vi "Settings Dialog.vi"(7 "Host":T1={"NI Software"=[{"ID"="ni-datasocket", "Version"="21.0.0.49352-0+f200"}, {"ID"="ni-vipm", "Version"="21.1.0.49472-0+f320"}, {"ID"="ni-labview-2021-core-x86-en", "Version"="21.1.2.49154-0+f2"}, {"ID"="ni-labview-2021-community-x86", "Version"="21.1.0.49478-0+f326"}, {"ID"="ni-labview-2021-database-toolkit-x86", "Version"="21.0.0.49154-0+f2"}, {"ID"="ni-labview-2021-datafinder-runtime-x86", "Version"="21.0.0.49153-0+f1"}, {"ID"="ni-labview-2021-datafinder-connectivity-x86", "Version"="21.0.0.49152-0+f0"}, {"ID"="ni-labview-2021-linx-toolkit-x86", "Version"="21.1.0.49152-0+f0"}, {"ID"="ni-labview-2021-report-generation-toolkit-x86", "Version"="21.0.0.49154-0+f2"}, {"ID"="ni-labview-2019-runtime-engine-x86", "Version"="19.1.5.49152-0+f0"}, {"ID"="ni-labview-2020-runtime-engine-x86", "Version"="20.1.1.49157-0+f5"}, {"ID"="ni-labview-2021-runtime-engine-x86", "Version"="21.1.2.49154-0+f2"}, {"ID"="ni-cvi-dotnet", "Version"="20.0.0.49152-0+f0"}, {"ID"="ni-cvi-analysis", "Version"="20.0.0.49152-0+f0"}, {"ID"="ni-cvi-networkstreams", "Version"="20.0.0.49152-0+f0"}, {"ID"="ni-cvi-network-variable", "Version"="20.0.0.49152-0+f0"}, {"ID"="ni-cvi-runtime-engine", "Version"="20.0.2.49152-0+f0"}, {"ID"="ni-cvi-rte", "Version"="20.0.2.49152-0+f0"}, {"ID"="ni-cvi-tdms", "Version"="20.0.1.49152-0+f0"}, {"ID"="mgi-solution-explorer", "Version"="2.5.0-53"}, {"ID"="ni-certificates", "Version"="21.5.0.49170-0+f18"}, {"ID"="ni-dataplugins-aop5", "Version"="19.5.0.7555-0+f2"}, {"ID"="ni-distributed-system-manager-2021", "Version"="21.0.0.49488-0+f336"}, {"ID"="ni-hardware-configuration-importer", "Version"="8.4.0.49152-0+f0"}, {"ID"="ni-labview-command-line-interface-x86", "Version"="4.0.0.49152-0+f0"}, {"ID"="ni-license-manager", "Version"="21.3.1.49163-0+f11"}, {"ID"="ni-max", "Version"="21.5.0.49391-0+f239"}, {"ID"="ni-package-manager", "Version"="23.0.0.49276-0+f124"}, {"ID"="ni-syscfg-dotnet-runtime", "Version"="21.5.0.49392-0+f240"}, {"ID"="ni-syscfg-runtime", "Version"="21.5.0.49392-0+f240"}, {"ID"="ni-syscfg-labview-2021-support-x86", "Version"="21.5.0.49392-0+f240"}, {"ID"="ni-system-webserver", "Version"="21.5.0.49152-0+f0"}, {"ID"="ni-update-service", "Version"="21.0.0.49243-0+f91"}, {"ID"="ni-usi-core", "Version"="21.5.0.49152-0+f0"}, {"ID"="ni-webserver", "Version"="21.3.0.49152-0+f0"}, {"ID"="ni-webservices-amqp-deployment-support-x86", "Version"="21.5.0.49152-0+f0"}, {"ID"="ni-webservices-amqp-labview-2021-support-x86", "Version"="21.5.0.49152-0+f0"}, {"ID"="ni-web-based-configuration", "Version"="21.5.0.49392-0+f240"}, {"ID"="ni-visa-runtime", "Version"="21.5.0.49252-0+f100"}, {"ID"="ni-variable-engine", "Version"="21.0.0.49350-0+f198"}], "IO Devices"=[]}, 8 "error in (no error)":errorcluster, 11 "Settings in":T13={"IO"={"Channel Settings"=[{"Name"="sim1", "Terminal Information"={"IO Device"=enum."none", "Channel"=0, "Sensor Type"=enum."Voltage"}, "Calibration Information"={"Excitation Voltage"=1.0, "Calibration Factor"=1.0, "Zero Value"=0.0, "Calibration Formula"="y = (x-x0) / (Ve * CF)", "Units"=""}}, {"Name"="sim2", "Terminal Information"={"IO Device"=enum."none", "Channel"=1, "Sensor Type"=enum."Voltage"}, "Calibration Information"={"Excitation Voltage"=1.0, "Calibration Factor"=1.0, "Zero Value"=0.0, "Calibration Formula"="(x-x0) / (Ve * CF)", "Units"=""}}, {"Name"="sim3", "Terminal Information"={"IO Device"=enum."none", "Channel"=2, "Sensor Type"=enum."Voltage"}, "Calibration Information"={"Excitation Voltage"=1.0, "Calibration Factor"=1.0, "Zero Value"=0.0, "Calibration Formula"="y = (x-x0) / (Ve * CF)", "Units"=""}}, {"Name"="sim4", "Terminal Information"={"IO Device"=enum."none", "Channel"=3, "Sensor Type"=enum."Voltage"}, "Calibration Information"={"Excitation Voltage"=1.0, "Calibration Factor"=1.0, "Zero Value"=0.0, "Calibration Formula"="(x-x0) / (Ve * CF)", "Units"=""}}], "Sensor Intervals"=[{"Interval"=enum."1 second", "Count"=1}], "Sensor Token"={"Next reading in ms"=0, "Interval Index"=0, "Interval Occurrence"=0}, "IO Context"={"Active Plugin"="", "API"=enum."Simulated", "API Wire"=variant}}, "Log"={"Path"=path "C:/dev/mux/git/github/lv-daq-app-template/data_log.csv", "Spreadsheet"=refnum, "Mode"=enum."Append"}, "Debug"={"Messages"=refnum}, "Graph Settings"={"Small Scale Max"=0.0, "Large Scale Max"=0.0, "Large Scale Threshold"=0.0}}) -> (0 "error out":errorcluster, 1 "Cancelled?":bool=TRUE, 3 "Settings out":T13={"IO"={"Channel Settings"=[{"Name"="sim1", "Terminal Information"={"IO Device"=enum."none", "Channel"=0, "Sensor Type"=enum."Voltage"}, "Calibration Information"={"Excitation Voltage"=1.0, "Calibration Factor"=1.0, "Zero Value"=0.0, "Calibration Formula"="y = (x-x0) / (Ve * CF)", "Units"=""}}, {"Name"="sim2", "Terminal Information"={"IO Device"=enum."none", "Channel"=1, "Sensor Type"=enum."Voltage"}, "Calibration Information"={"Excitation Voltage"=1.0, "Calibration Factor"=1.0, "Zero Value"=0.0, "Calibration Formula"="(x-x0) / (Ve * CF)", "Units"=""}}, {"Name"="sim3", "Terminal Information"={"IO Device"=enum."none", "Channel"=2, "Sensor Type"=enum."Voltage"}, "Calibration Information"={"Excitation Voltage"=1.0, "Calibration Factor"=1.0, "Zero Value"=0.0, "Calibration Formula"="y = (x-x0) / (Ve * CF)", "Units"=""}}, {"Name"="sim4", "Terminal Information"={"IO Device"=enum."none", "Channel"=3, "Sensor Type"=enum."Voltage"}, "Calibration Information"={"Excitation Voltage"=1.0, "Calibration Factor"=1.0, "Zero Value"=0.0, "Calibration Formula"="(x-x0) / (Ve * CF)", "Units"=""}}], "Sensor Intervals"=[{"Interval"=enum."1 second", "Count"=1}], "Sensor Token"={"Next reading in ms"=0, "Interval Index"=0, "Interval Occurrence"=0}, "IO Context"={"Active Plugin"="", "API"=enum."Simulated", "API Wire"=variant}}, "Log"={"Path"=path "C:/dev/mux/git/github/lv-daq-app-template/data_log.csv", "Spreadsheet"=refnum, "Mode"=enum."Append"}, "Debug"={"Messages"=refnum}, "Graph Settings"={"Small Scale Max"=0.0, "Large Scale Max"=0.0, "Large Scale Threshold"=0.0}})   [LabVIEW 2021, in "Settings.lvlib"]
doc: "Dialog for selecting user specified settings."
uses:
  Settings.lvlib
  Settings.ctl
  Acquisition/Hardware Configuration.ctl
  Acquisition/Channel Settings.ctl
  Acquisition/IO Device.ctl
  Acquisition/Sensor Type.ctl
  Interval Timer/Repeat Interval.ctl
  Interval Timer/Interval Length.ctl
  Interval Timer/Interval Token.ctl
  Acquisition/IO Context.ctl
  Acquisition/IO API.ctl
  Logging/Logging Configuration.ctl
  Logging/Logging Mode.ctl
  Diagnostics/Diagnostics Configuration.ctl
  controls/Graph Settings.ctl
  Acquisition/Host Resources.ctl
  Acquisition/Host Software Package.ctl
  Acquisition/Host IO Resource.ctl
  Logging/Logging.lvlib
  Acquisition/Acquisition.lvlib
  Diagnostics/Diagnostics.lvlib
  Interval Timer/Interval Timer.lvlib
panel:
  in  "IO tab control":T4(tab)
  in  "Channel Settings":T7(array[cluster])
  in  "Calibration Settings":T8(array[cluster])
  in  "New x0 Button":bool
  out "x0":dbl=nan
  out "CF":dbl=nan
  out "Vex":dbl=nan
  out "Preview Chart":waveform(dbl)(graph)={"t0"=timestamp(3763062488.961019 s since 1904-01-01), "dt"=1.0, "Y"=[3.134800048306457], "attributes"=variant("NI_ChannelName"=variant(string "sim1"))}
  in  "Channel to Preview":string(combo)
  in  "Stop Preview Button":bool
  in  "Start Preview Button":bool
  in  "Active Plugin":string(combo)
  in  "Graph settings":T9
  in  "Sensor Intervals":T10[](array[typedef])=[{"Interval"=enum."1 second", "Count"=1}]
  out "Host out":T1
  in  "Log File tab control":T12(tab)=enum."Append to existing log"
  in  "Refresh Button":bool
  in  "New log file path":path=path "C:/dev/mux/git/github/lv-daq-app-template/data_log.csv"
  in  "Existing log file path":string="C:\\dev\\mux\\git\\github\\lv-daq-app-template\\data_log.csv"
  in  "Autoname new log path":string="C:\\dev\\mux\\git\\github\\lv-daq-app-template\\data_log.csv"
  in  "Cancel Button":bool
  in  "OK Button":bool
  # "Non visible portion of dialog (needed for connector pane)."
  # "Method: (x-x0) / (Ve * CF)"
  # "Method: (x-x0) / (Ve * CF)"
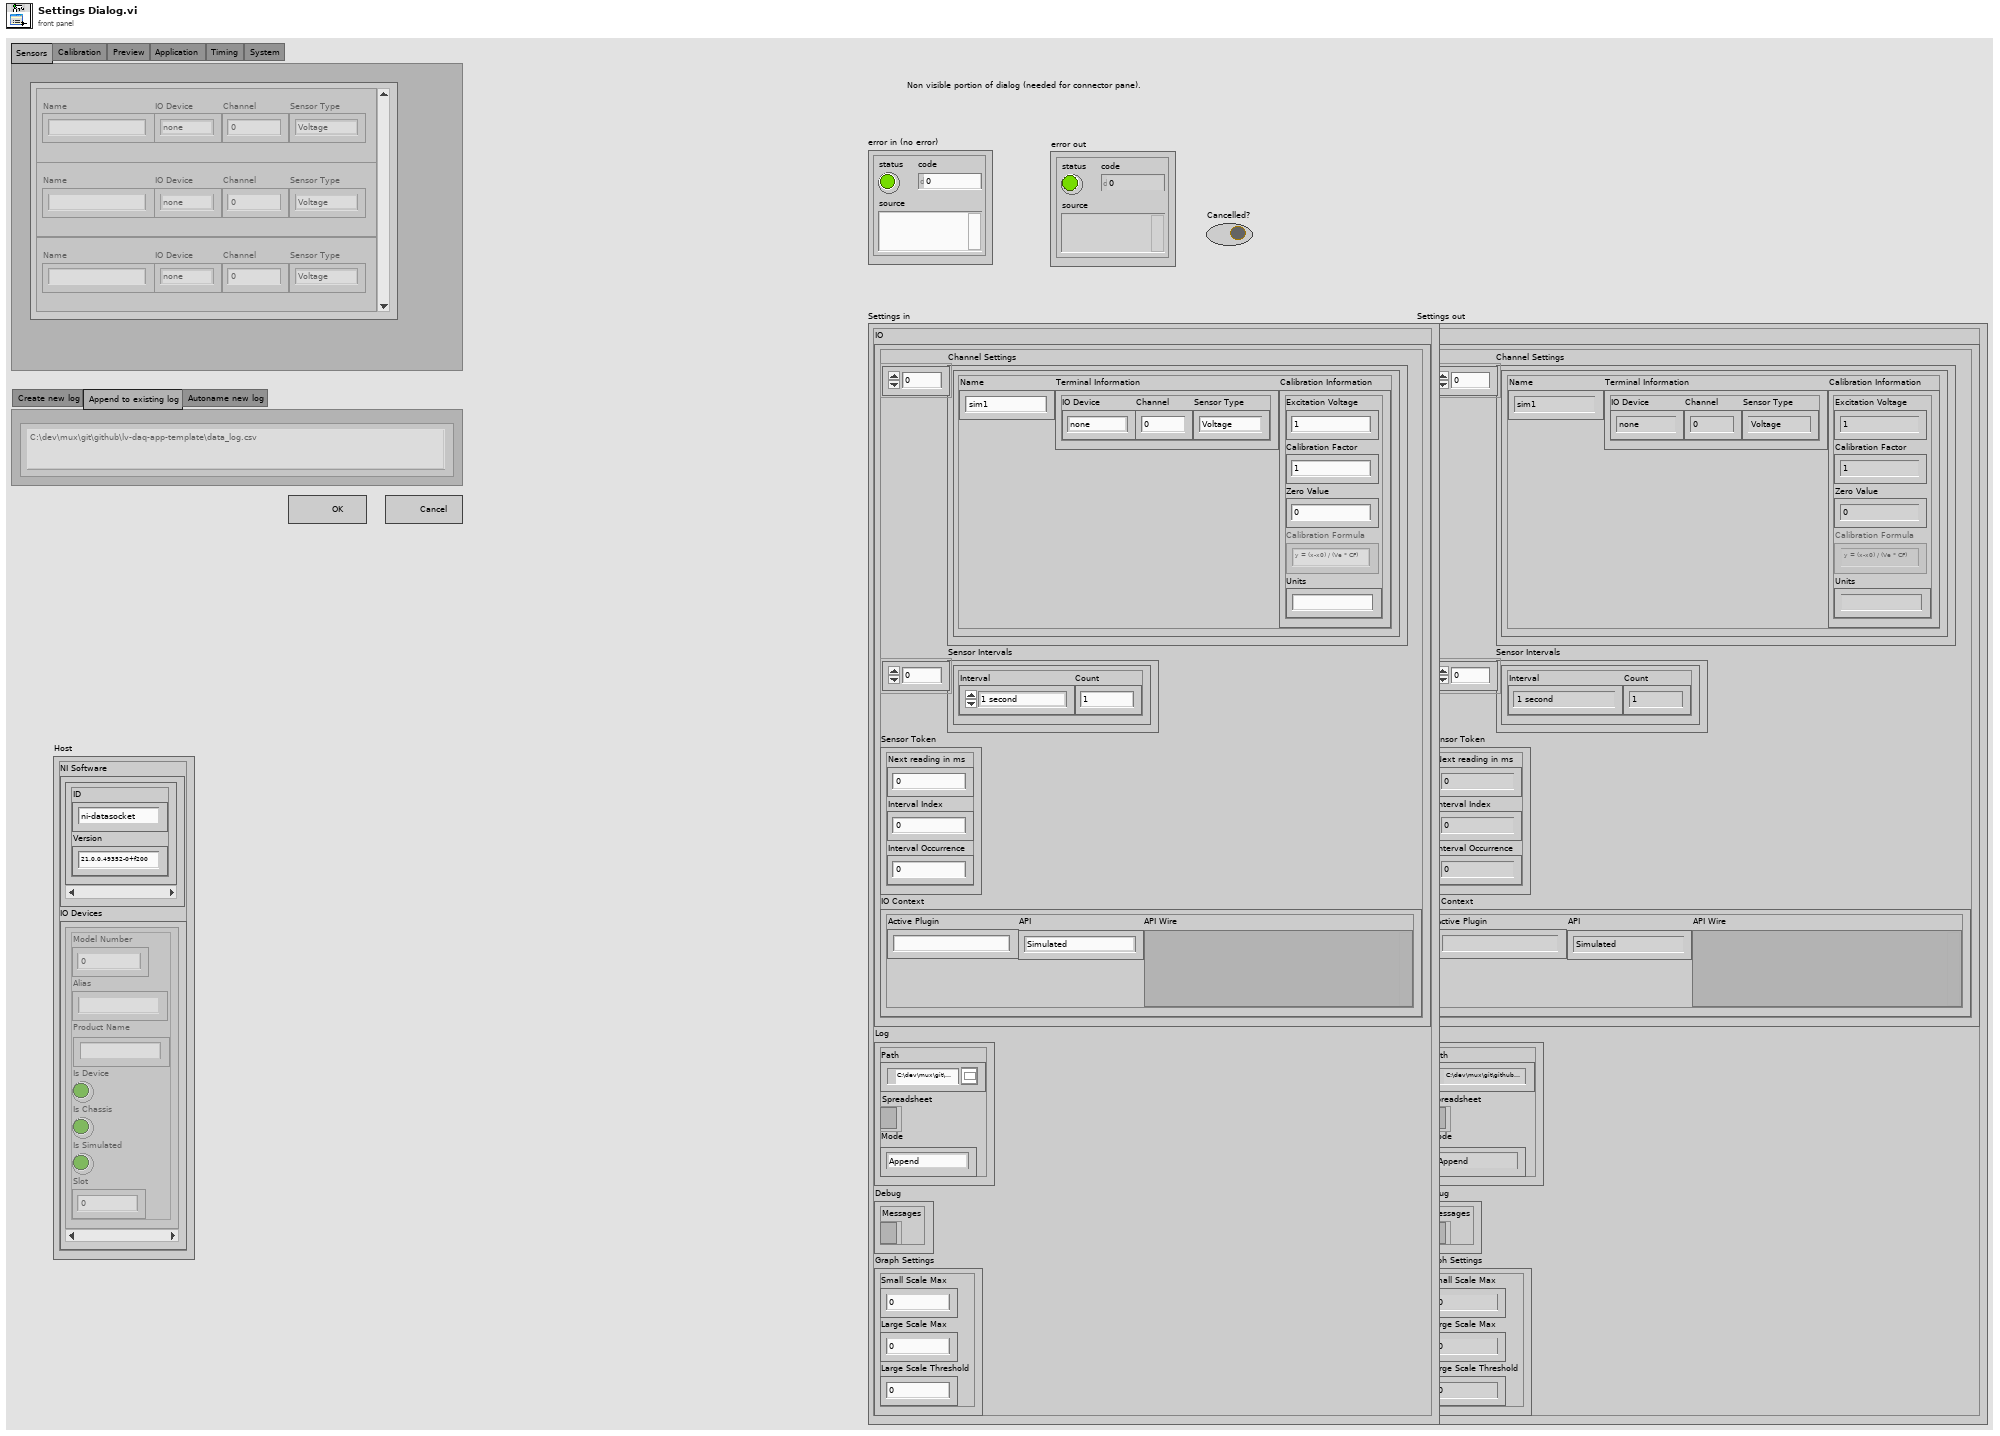
[diagram p1: front panel]
types:
  T1 = typedef "Acquisition.lvlib/Host Resources.ctl" = cluster{"NI Software":T2[], "IO Devices":T3[]}
  T2 = typedef "Acquisition.lvlib/Host Software Package.ctl" = cluster{"ID":string, "Version":string}
  T3 = typedef "Acquisition.lvlib/Host IO Resource.ctl" = cluster{"Model Number":u32, "Alias":string, "Product Name":string, "Is Device":bool, "Is Chassis":bool, "Is Simulated":bool, "Slot":i32}
  T4 = enum32{"Sensors", "Calibration", "Preview", "Application", "Timing", "System"}
  T5 = typedef "Acquisition.lvlib/IO Device.ctl" = enum16{"none", "9219", "9401"}
  T6 = typedef "Acquisition.lvlib/Sensor Type.ctl" = enum16{"Voltage", "Load", "Pressure", "Encoder"}
  T7 = cluster{"Name":string, "Terminal Information":cluster{"IO Device":T5, "Channel":i32, "Sensor Type":T6}}[]
  T8 = cluster{"Name":string, "Calibration Information":cluster{"Excitation":dbl, "Cal. Factor":dbl, "Zero Value":dbl, "Units":string}}[]
  T9 = cluster{"Small Scale Maximum":dbl, "Large Scale Threshold":dbl, "Large Scale Maximum":dbl}
  T10 = typedef "Interval Timer.lvlib/Repeat Interval.ctl" = cluster{"Interval":T11, "Count":i32}
  T11 = typedef "Interval Timer.lvlib/Interval Length.ctl" = enum16{"Manual control", "1 second", "10 seconds", "30 seconds", "60 seconds", "600 seconds", "1200 seconds", "3600 seconds"}
  T12 = enum32{"Create new log", "Append to existing log", "Autoname new log"}
  T13 = typedef "Settings.lvlib/Settings.ctl" = cluster{"IO":T14, "Log":T19, "Debug":T21, "Graph Settings":T22}
  T14 = typedef "Acquisition.lvlib/Hardware Configuration.ctl" = cluster{"Channel Settings":T15[], "Sensor Intervals":T10[], "Sensor Token":T16, "IO Context":T17}
  T15 = typedef "Acquisition.lvlib/Channel Settings.ctl" = cluster{"Name":string, "Terminal Information":cluster{"IO Device":T5, "Channel":i32, "Sensor Type":T6}, "Calibration Information":cluster{"Excitation Voltage":dbl, "Calibration Factor":dbl, "Zero Value":dbl, "Calibration Formula":string, "Units":string}}
  T16 = typedef "Interval Timer.lvlib/Interval Token.ctl" = cluster{"Next reading in ms":u32, "Interval Index":i32, "Interval Occurrence":i32}
  T17 = typedef "Acquisition.lvlib/IO Context.ctl" = cluster{"Active Plugin":string, "API":T18, "API Wire":variant}
  T18 = typedef "Acquisition.lvlib/IO API.ctl" = enum16{"Simulated", "DAQmx"}
  T19 = typedef "Logging.lvlib/Logging Configuration.ctl" = cluster{"Path":path, "Spreadsheet":refnum<file>, "Mode":T20}
  T20 = typedef "Logging.lvlib/Logging Mode.ctl" = enum16{"Overwrite", "Append", "Create New"}
  T21 = typedef "Diagnostics.lvlib/Diagnostics Configuration.ctl" = cluster{"Messages":refnum<file>}
  T22 = typedef "Graph Settings.ctl" = cluster{"Small Scale Max":dbl, "Large Scale Max":dbl, "Large Scale Threshold":dbl}
  T23 = cluster{"Name":string, "Calibration Information":cluster{"Excitation Voltage":dbl, "Calibration Factor":dbl, "Zero Value":dbl, "Units":string}}[]
  T24 = typedef "Acquisition.lvlib/Acquired Data.ctl" = cluster{"Waveform Array":waveform(dbl)[]}
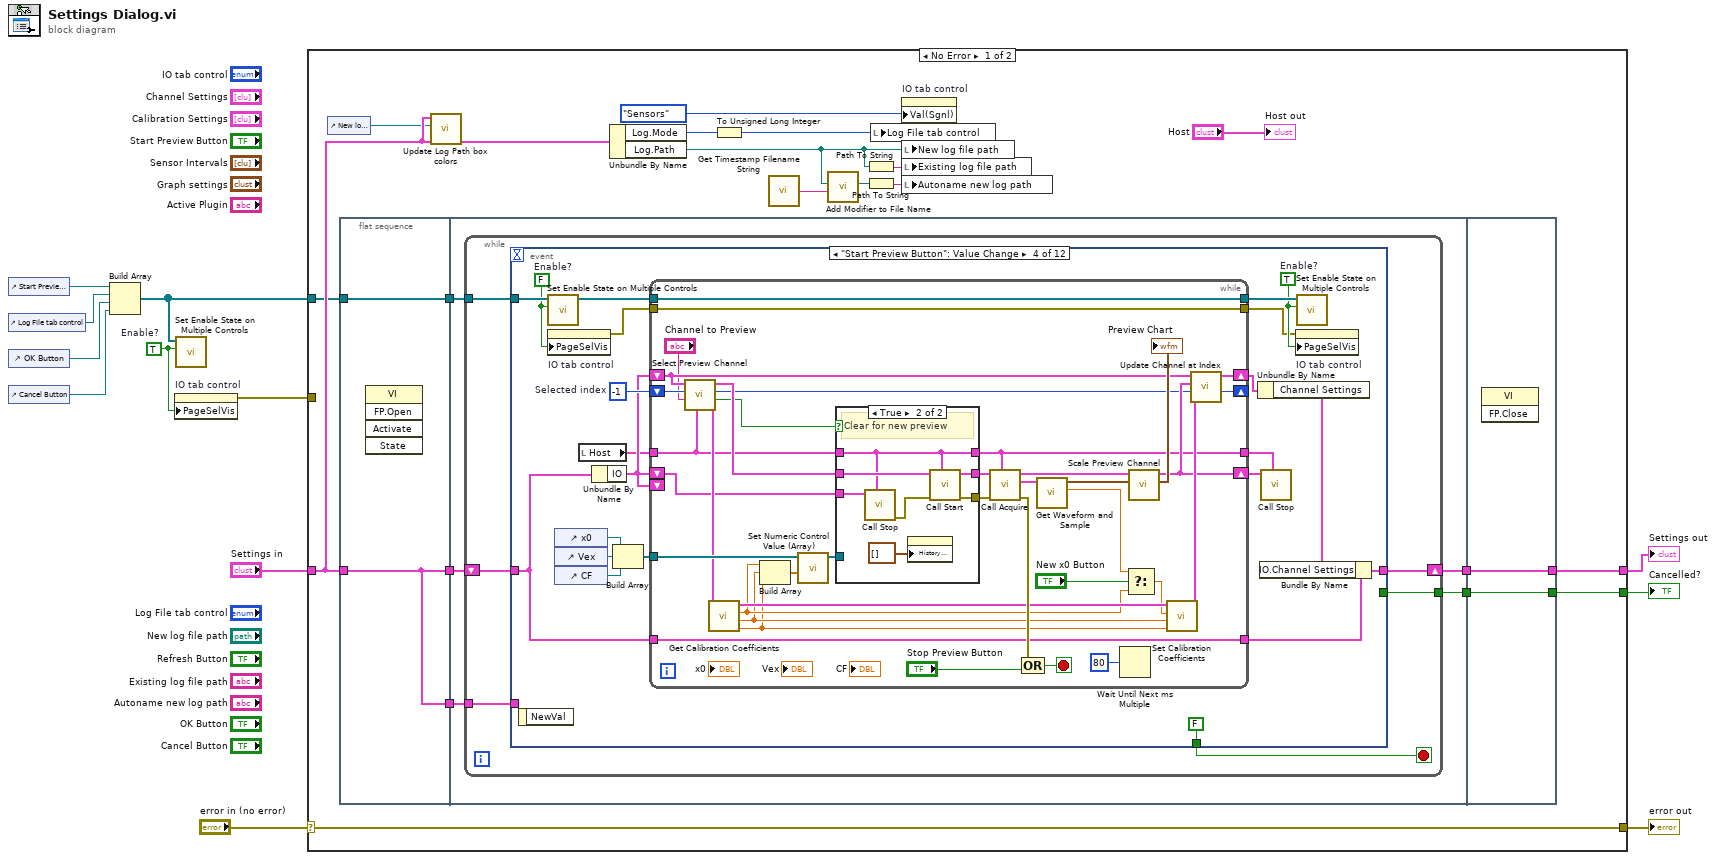
[diagram p0: block diagram]
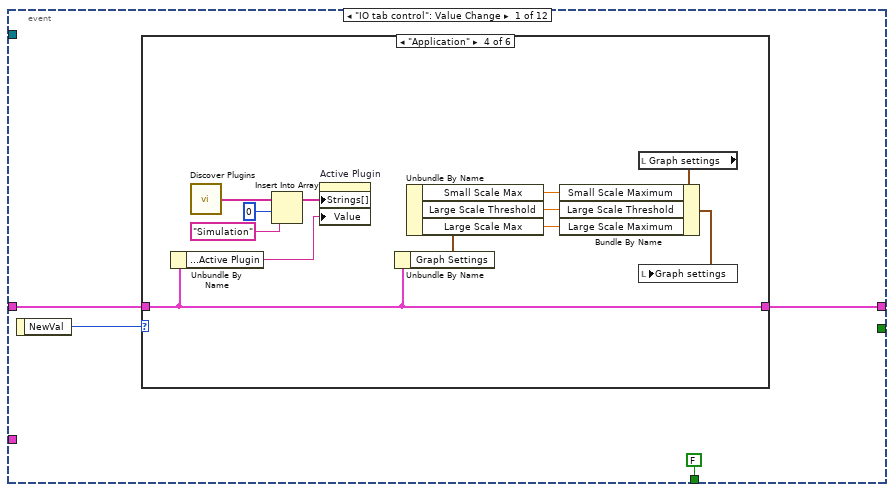
[diagram p2: hidden frame]
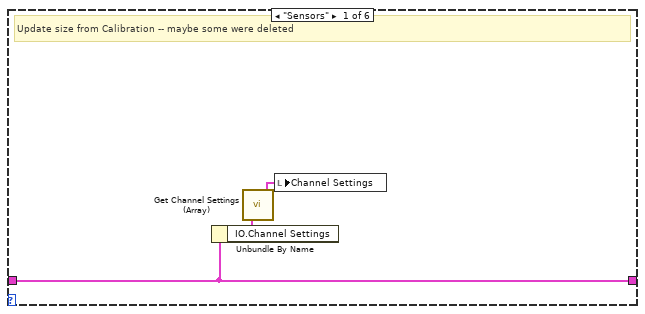
[diagram p3: hidden frame]
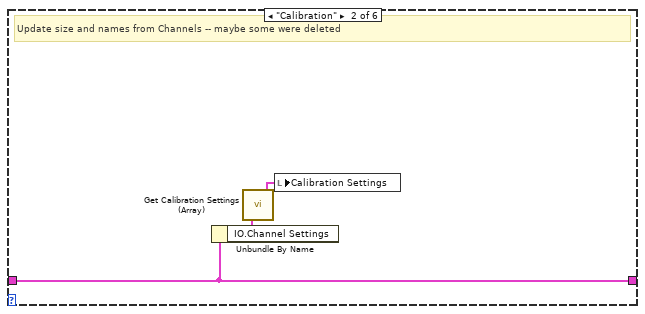
[diagram p4: hidden frame]
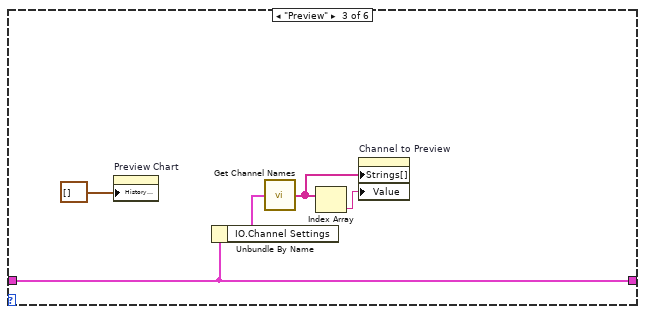
[diagram p5: hidden frame]
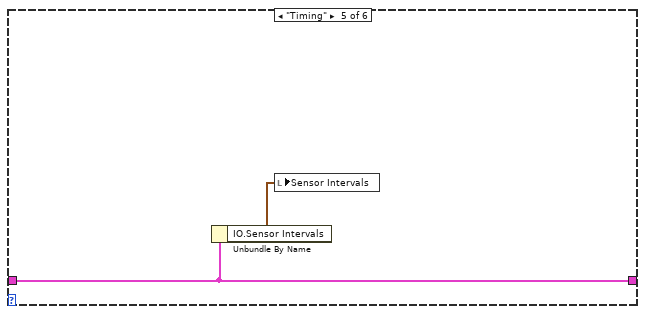
[diagram p6: hidden frame]
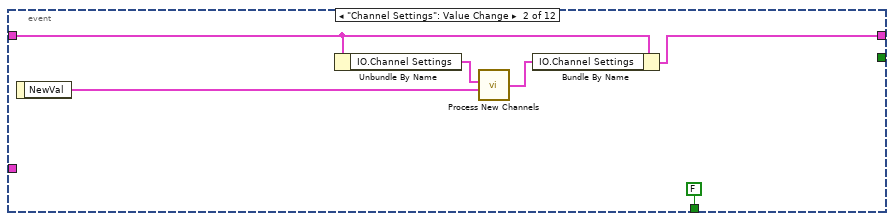
[diagram p8: hidden frame]
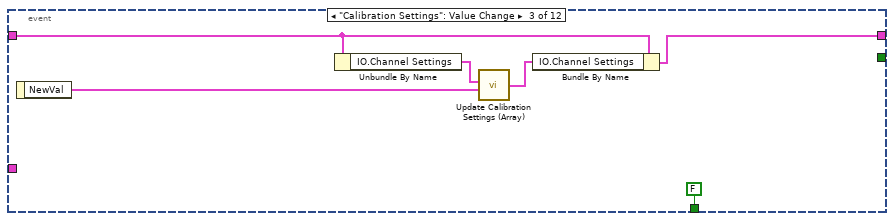
[diagram p9: hidden frame]
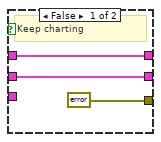
[diagram p10: hidden frame]
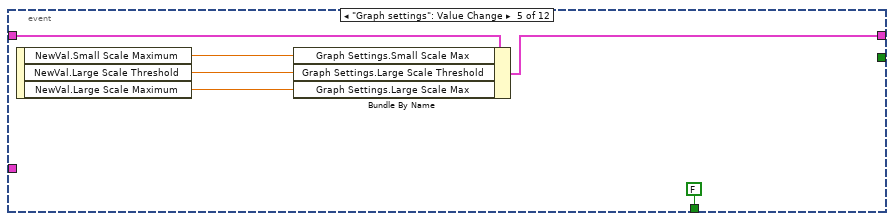
[diagram p11: hidden frame]
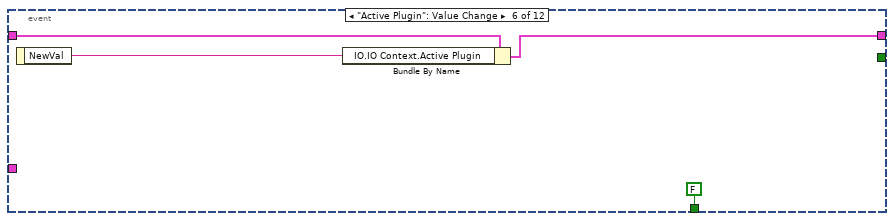
[diagram p12: hidden frame]
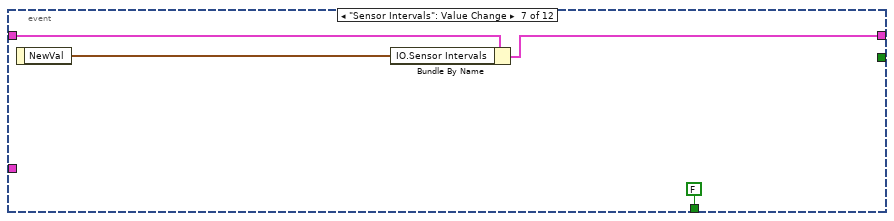
[diagram p13: hidden frame]
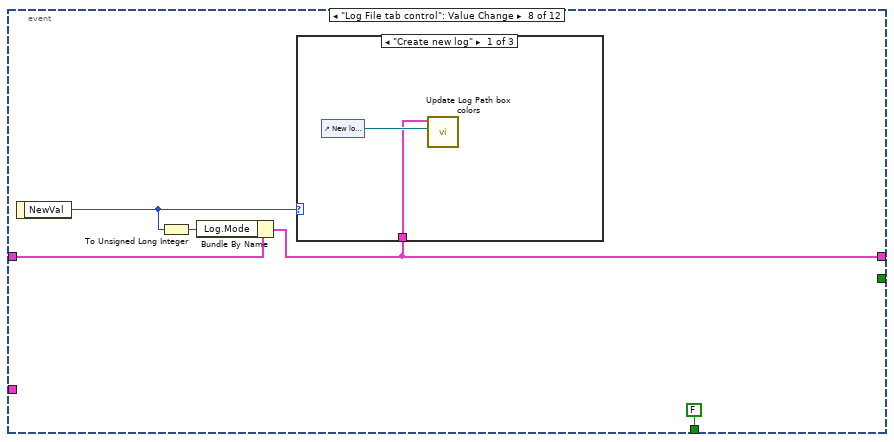
[diagram p14: hidden frame]
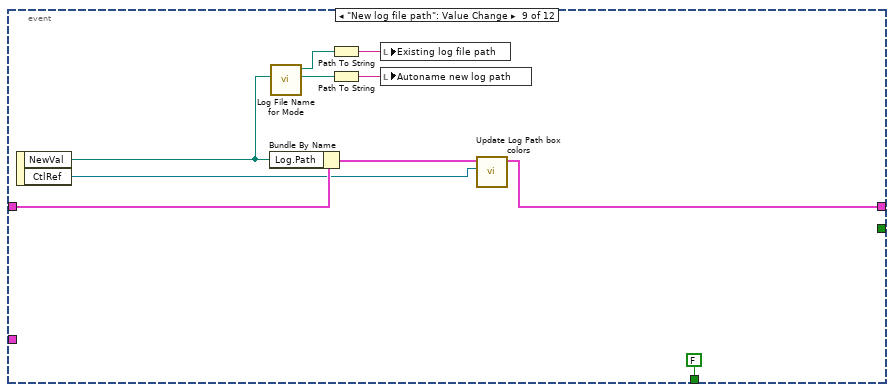
[diagram p17: hidden frame]
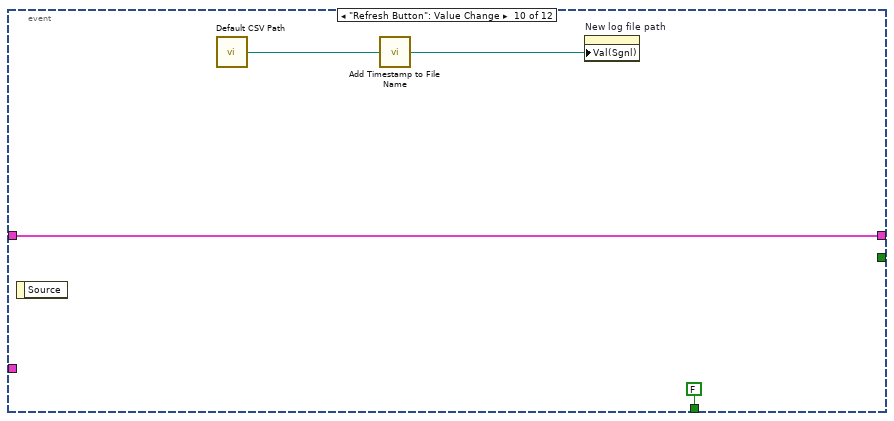
[diagram p18: hidden frame]
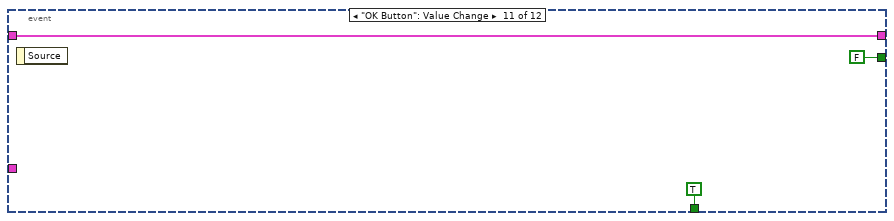
[diagram p19: hidden frame]
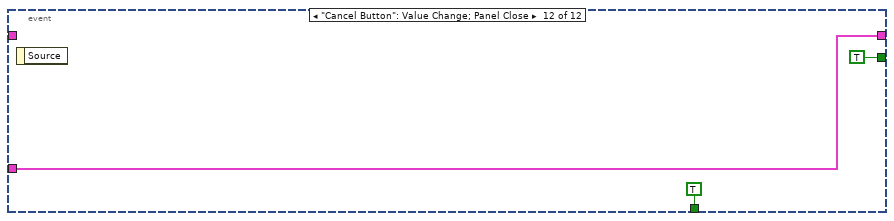
[diagram p20: hidden frame]
diagram:
  w2 = TRUE  # Enable?
  n1 = control-ref of="Start Preview Button"() -> (w7:refnum<vi>)
  n2 = control-ref of="Log File tab control"() -> (w6:refnum<vi>)
  n3 = control-ref of="OK Button"() -> (w5:refnum<vi>)
  n4 = control-ref of="Cancel Button"() -> (w4:refnum<vi>)
  n5 = Build Array(w7, w6, w5, w4) -> (w3:refnum<vi>[])
  n6 = property on="IO tab control" class="TabCtl (strict)"("PageSelVis"=w2) -> (error out=w1:errorcluster)  [unwired: 2 in, 1 out]
  n7 = call "Set Enable State on Multiple Controls.vi"("Enable?"=w2, "Controls"=w3) -> ()  [unwired: 9 in, 1 out]
  n8 = case shown="No Error" "error in (no error)" {
    selector: "error in (no error)" -> [w32 w202]
    tunnel: [w32 w202] -> w11
    tunnel: "Settings in" -> [w25 w201]
    tunnel: [w31 w201] -> w9
    tunnel: [w26 TRUE ("UI Refresh Needed?")] -> w8
    tunnel: w3 -> [w22 _]
    tunnel: w1 -> [_ _]
    frame No Error {
      n9 = control-ref of="New log file path"() -> (w24:refnum<vi>)
      n10 = flat-sequence {
        tunnel: w25 -> [w33]
        tunnel: [w33] -> w30
        tunnel: [w34] -> w23
        tunnel: w22 -> [w34]
        tunnel: [w33] -> w15
        tunnel: w30 -> [w37]
        tunnel: [w39] -> w29
        tunnel: [w38] -> w28
        tunnel: w23 -> [w36]
        tunnel: w15 -> [w35]
        tunnel: [w198] -> w31
        tunnel: [w199] -> w26
        tunnel: w29 -> [w199]
        tunnel: w28 -> [w198]
        frame #0 {
          n11 = invoke class="VI" method="FP.Open"() -> ()  [unwired: 5 in, 5 out]
        }
        frame #1 {
          n12 = while {
            tunnel: [w45] -> w39
            shift-right: [w44] -> w38
            shift-left: w37 -> [w40]
            tunnel: w36 -> [w42]
            tunnel: w35 -> [w41]
            stop <- w43 stop-if-true
            n13 = event shown="[3] \"Start Preview Button\": Value Change" {
              selector: _ -> [_ _ _ _ _ _ _ _ _ _ _ _]
              dyn-events: _ -> [_ _ _ _ _ _ _ _ _ _ _ _]
              timeout: _ -> [_ _ _ _ _ _ _ _ _ _ _ _]
              tunnel: [w47 w79 w85 w90 w161 w164 w169 w174 w186 w191 w192 w195] -> w44
              tunnel: w40 -> [w48 w80 w86 w94 w162 w166 w170 w175 w187 w191 w192 _]
              tunnel: [_ _ _ _ _ _ _ _ _ _ FALSE ("UI Refresh Needed?") TRUE ("UI Refresh Needed?")] -> w45
              tunnel: [FALSE ("UI Refresh Needed?") FALSE ("UI Refresh Needed?") FALSE ("UI Refresh Needed?") FALSE ("UI Refresh Needed?") FALSE ("UI Refresh Needed?") FALSE ("UI Refresh Needed?") FALSE ("UI Refresh Needed?") FALSE ("UI Refresh Needed?") FALSE ("UI Refresh Needed?") FALSE ("UI Refresh Needed?") TRUE ("UI Refresh Needed?") TRUE ("UI Refresh Needed?")] -> w43
              tunnel: w42 -> [_ _ _ w108 _ _ _ _ _ _ _ _]
              tunnel: w41 -> [_ _ _ _ _ _ _ _ _ _ _ w195]
              event "IO tab control": Value Change {
                n14 = event-data() -> ("NewVal"=w49:T4)  [unwired: 1 in]
                n15 = case shown="\"Application\"" w49 {
                  tunnel: w48 -> [w51 w55 w60 w62 w74 w75]
                  tunnel: [w51 w55 w60 w62 w74 w75] -> w47
                  frame "Sensors" {
                    # "Update size from Calibration -- maybe some were deleted"
                    n16 = Unbundle By Name(w51) -> ("IO.Channel Settings"=w50:T15[])
                    n17 = call "Get Channel Settings (Array).vi"("Channel Settings typedef"=w50) -> ("Channel Settings ducktype"=w52:T7)
                    n18 = local write "Channel Settings"(w52) -> ()
                  }
                  frame "Calibration" {
                    # "Update size and names from Channels -- maybe some were deleted"
                    n19 = Unbundle By Name(w55) -> ("IO.Channel Settings"=w54:T15[])
                    n20 = call "Get Calibration Settings (Array).vi"("Channel Settings typedef"=w54) -> ("Calibration Settings ducktype"=w53:T23)
                    n21 = local write "Calibration Settings"(w53) -> ()
                  }
                  frame "Preview" {
                    n22 = property on="Preview Chart" class="WFChart (strict)"("History Data"=waveform(dbl)[] []) -> ()  [unwired: 2 in, 2 out]
                    n23 = Unbundle By Name(w60) -> ("IO.Channel Settings"=w59:T15[])
                    n24 = call "Get Channel Names.vi"("Channel Settings"=w59) -> ("Channel Names"=w58:string[])
                    n25 = Index Array(array=w58) -> (element=w57:string)  [unwired: 1 in]
                    n26 = property on="Channel to Preview" class="CmbBox"("Strings[]"=w58, "Value"=w57) -> ()  [unwired: 2 in, 2 out]
                  }
                  frame "Application" {
                    n27 = Unbundle By Name(w62) -> ("IO.IO Context.Active Plugin"=w61:string)
                    n28 = call "Discover Plugins.vi"() -> ("plugins"=w63:string[])
                    n29 = Insert Into Array(array=w63, index=0, new element="Simulation" ("new element/subarray")) -> (w66:string[])
                    n30 = property on="Active Plugin" class="CmbBox"("Strings[]"=w66, "Value"=w61) -> ()  [unwired: 2 in, 2 out]
                    n31 = Unbundle By Name(w62) -> ("Graph Settings"=w70:T22)
                    n32 = Unbundle By Name(w70) -> ("Small Scale Max"=w69:dbl, "Large Scale Threshold"=w68:dbl, "Large Scale Max"=w67:dbl)
                    n33 = local read "Graph settings"() -> (w72:T9)
                    n34 = Bundle By Name(cluster=w72, "Small Scale Maximum"=w69, "Large Scale Threshold"=w68, "Large Scale Maximum"=w67) -> (w71:T9)
                    n35 = local write "Graph settings"(w71) -> ()
                  }
                  frame "Timing" {
                    n36 = Unbundle By Name(w74) -> ("IO.Sensor Intervals"=w73:T10[])
                    n37 = local write "Sensor Intervals"(w73) -> ()
                  }
                  frame "System" {
                  }
                }
              }
              event "Channel Settings": Value Change {
                n38 = event-data() -> ("NewVal"=w76:T7)  [unwired: 1 in]
                n39 = Unbundle By Name(w80) -> ("IO.Channel Settings"=w78:T15[])
                n40 = call "Process New Channels.vi"("Channel Settings ducktype"=w76, "Channel Settings in"=w78) -> ("Channel Settings out"=w77:T15[])  [unwired: 2 in]
                n41 = Bundle By Name(cluster=w80, "IO.Channel Settings"=w77) -> (w79:T13)
              }
              event "Calibration Settings": Value Change {
                n42 = event-data() -> ("NewVal"=w82:T8)  [unwired: 1 in]
                n43 = Unbundle By Name(w86) -> ("IO.Channel Settings"=w84:T15[])
                n44 = call "Update Calibration Settings (Array).vi"("Calibration Settings ducktype"=w82, "Channel Settings in"=w84) -> ("Channel Settings out"=w83:T15[])  [unwired: 2 in]
                n45 = Bundle By Name(cluster=w86, "IO.Channel Settings"=w83) -> (w85:T13)
              }
              event "Start Preview Button": Value Change {
                w101 = -1  # Selected index
                w103 = TRUE  # Enable?
                w104 = FALSE  # Enable?
                n46 = event-data() -> ()  [unwired: 1 in, 1 out]
                n47 = call "Set Enable State on Multiple Controls.vi"("Enable?"=w104, "Controls"=w108) -> ("Controls dup"=w107:refnum<vi>[])  [unwired: 9 in]
                n48 = property on="IO tab control" class="TabCtl (strict)"("PageSelVis"=w104) -> (error out=w105:errorcluster)  [unwired: 2 in, 1 out]
                n49 = control-ref of="x0"() -> (w98:refnum<vi>)
                n50 = control-ref of="Vex"() -> (w100:refnum<vi>)
                n51 = control-ref of="CF"() -> (w97:refnum<vi>)
                n52 = local read "Host"() -> (w92:T1)
                n53 = Unbundle By Name(w94) -> ("IO"=w93:T14)
                n54 = Build Array(w98, w100, w97) -> (w99:refnum<vi>[])
                n55 = while {
                  tunnel: w107 -> [w144]
                  tunnel: [w144] -> w106
                  tunnel: w105 -> [w143]
                  tunnel: [w143] -> w102
                  shift-right: [w138] -> _
                  shift-left: w101 -> [w113]
                  shift-right: [w122] -> w96
                  shift-left: w93 -> [_]
                  tunnel: w94 -> [w115]
                  tunnel: [w115] -> w91
                  tunnel: w99 -> [w137]
                  shift-left: w93 -> [w129]
                  shift-right: [w127] -> w89
                  shift-left: w93 -> [w126]
                  tunnel: [w121] -> w95
                  tunnel: w92 -> [w114]
                  stop <- w124 stop-if-true
                  n56 = call "Select Preview Channel.vi"("Host Resources in"=w114, "Channel to Preview"="Channel to Preview", "Previous Selected Channel"=w113, "Hardware Configuration"=w126) -> ("Selected Channel"=w134:T15, "Selected Channel Changed?"=w111:bool, "Selected Channel Index"=w120:i32, "Hardware Configuration for Preview Channel"=w140:T14)  [unwired: 4 in]
                  n57 = call "Get Calibration Coefficients.vi"("Channel Settings"=w134) -> ("Calibration Factor"=w116:dbl, "Excitation Voltage"=w117:dbl, "Zero Value"=w118:dbl, "Channel Settings out"=w119:T15)  [unwired: 7 in]
                  n58 = Build Array(w118, w117, w116) -> (w135:dbl[])
                  n59 = call "Set Numeric Control Value (Array).vi"("New values"=w135, "Digital Contol refs"=w137) -> ("Digital Control refs out"=w136:refnum<vi>[])  [unwired: 8 in, 1 out]
                  n60 = case shown="True" w111 {
                    tunnel: w140 -> [w149 w155]
                    tunnel: w136 -> [_ _]
                    tunnel: [w149 w154] -> w133
                    tunnel: w114 -> [w148 w151]
                    tunnel: w129 -> [_ w153]
                    tunnel: [w148 w151] -> w121
                    tunnel: [errorcluster {"status"=FALSE, "code"=0, "source"=""} ("error out") w150] -> w125
                    frame False {
                      # "Keep charting"
                    }
                    frame True {
                      # "Clear for new preview"
                      n61 = call "Call Stop.vi"("Host Resources"=w151, "Hardware Configuration in"=w153) -> ("error out"=w152:errorcluster)  [unwired: 8 in, 1 out]
                      n62 = property on="Preview Chart" class="WFChart (strict)"("History Data"=waveform(dbl)[] []) -> ()  [unwired: 2 in, 2 out]
                      n63 = call "Call Start.vi"("Host Resources"=w151, "error in (no error)"=w152, "Hardware Configuration in"=w155) -> ("error out"=w150:errorcluster, "Hardware Configuration out"=w154:T14)  [unwired: 7 in]
                    }
                  }
                  n64 = call "Call Acquire.vi"("Host Resources"=w121, "error in (no error)"=w125, "Hardware Configuration in"=w133) -> ("error out"=w123:errorcluster, "Acquired Data"=w132:T24, "Hardware Configuration out"=w130:T14)  [unwired: 6 in]
                  n65 = Compound Arithmetic op=OR(w123, "Stop Preview Button") -> (w124:bool)
                  n66 = call "Get Waveform and Sample.vi"("Acquired Data"=w132) -> ("As scalar"=w141:dbl, "Waveform"=w131:waveform(dbl))  [unwired: 9 in]
                  n67 = Wait Until Next ms Multiple(millisecond multiple=u32 80 ("Loop Wait (ms)")) -> ()  [unwired: 1 out]
                  n68 = Select(t=w141, s="New x0 Button", f=w118) -> (s? t:f=w110:dbl)
                  n69 = call "Scale Preview Channel.vi"("Waveform"=w131, "Hardware Configuration in"=w130) -> ("Scaled waveform"=→"Preview Chart":waveform(dbl), "Hardware Configuration in out"=w122:T14)  [unwired: 7 in, 1 out]
                  n70 = call "Set Calibration Coefficients.vi"("Calibration Factor"=w116, "Excitation Voltage"=w117, "Zero Value"=w110, "Channel Settings"=w119) -> ("Updated Channel Settings"=w139:T15)  [unwired: 7 in]
                  n71 = call "Update Channel at Index.vi"("Updated Channel Settings"=w139, "Updated Channel Index"=w120, "Hardware Configuration from Preview Channel"=w122, "Hardware Configuration"=w126) -> ("Updated Channel Index out"=w138:i32, "Hardware Configuration out"=w127:T14)  [unwired: 6 in]
                }
                n72 = Unbundle By Name(w89) -> ("Channel Settings"=w88:T15[])
                n73 = Bundle By Name(cluster=w91, "IO.Channel Settings"=w88) -> (w90:T13)
                n74 = call "Call Stop.vi"("Host Resources"=w95, "Hardware Configuration in"=w96) -> ()  [unwired: 8 in, 2 out]
                n75 = property on="IO tab control" class="TabCtl (strict)"(error in=w102, "PageSelVis"=w103) -> ()  [unwired: 1 in, 2 out]
                n76 = call "Set Enable State on Multiple Controls.vi"("Enable?"=w103, "Controls"=w106) -> ()  [unwired: 9 in, 1 out]
              }
              event "Graph settings": Value Change {
                n77 = event-data() -> ("NewVal.Small Scale Maximum"=w160:dbl, "NewVal.Large Scale Threshold"=w159:dbl, "NewVal.Large Scale Maximum"=w158:dbl)  [unwired: 1 in]
                n78 = Bundle By Name(cluster=w162, "Graph Settings.Small Scale Max"=w160, "Graph Settings.Large Scale Threshold"=w159, "Graph Settings.Large Scale Max"=w158) -> (w161:T13)
              }
              event "Active Plugin": Value Change {
                n79 = event-data() -> ("NewVal"=w165:string)  [unwired: 1 in]
                n80 = Bundle By Name(cluster=w166, "IO.IO Context.Active Plugin"=w165) -> (w164:T13)
              }
              event "Sensor Intervals": Value Change {
                n81 = event-data() -> ("NewVal"=w168:T10[])  [unwired: 1 in]
                n82 = Bundle By Name(cluster=w170, "IO.Sensor Intervals"=w168) -> (w169:T13)
              }
              event "Log File tab control": Value Change {
                n83 = event-data() -> ("NewVal"=w172:T12)  [unwired: 1 in]
                n84 = To Unsigned Long Integer(number=w172) -> (unsigned 32bit integer=w171:u32)
                n85 = Bundle By Name(cluster=w175, "Log.Mode"=w171) -> (w174:T13)
                n86 = case shown="\"Create new log\"" w172 {
                  tunnel: w174 -> [w176 _ _]
                  frame "Create new log" {
                    n87 = control-ref of="New log file path"() -> (w177:refnum<vi>)
                    n88 = call "Update Log Path box colors.vi"("Path Ref"=w177, "Settings in"=w176) -> ()  [unwired: 8 in, 2 out]
                  }
                  frame "Append to existing log" {
                  }
                  frame "Autoname new log" {
                  }
                }
              }
              event "New log file path": Value Change {
                n89 = event-data() -> ("NewVal"=w179:path, "CtlRef"=w183:refnum<vi>)  [unwired: 1 in]
                n90 = Bundle By Name(cluster=w187, "Log.Path"=w179) -> (w184:T13)
                n91 = call "Log File Name for Mode.vi"("base path"=w179) -> ("for Create New"=w180:path, "for Append"=w178:path)  [unwired: 6 in, 3 out]
                n92 = Path To String(path=w178) -> (string=w185:string)
                n93 = Path To String(path=w180) -> (string=w181:string)
                n94 = local write "Existing log file path"(w185) -> ()
                n95 = local write "Autoname new log path"(w181) -> ()
                n96 = call "Update Log Path box colors.vi"("Path Ref"=w183, "Settings in"=w184) -> ("Settings out"=w186:T13)  [unwired: 8 in, 1 out]
              }
              event "Refresh Button": Value Change {
                n97 = event-data() -> ()  [unwired: 1 in, 1 out]
                n98 = call "Default CSV Path.vi"() -> ("CSV file path"=w190:path)
                n99 = call "Add Timestamp to File Name.vi"("base path"=w190) -> ("timestamped path"=w188:path)
                n100 = property on="New log file path" class="Path"("Val(Sgnl)"=w188) -> ()  [unwired: 2 in, 2 out]
              }
              event "OK Button": Value Change {
                n101 = event-data() -> ()  [unwired: 1 in, 1 out]
              }
              event "Cancel Button": Value Change; Panel Close {
                n102 = event-data() -> ()  [unwired: 1 in, 1 out]
              }
            }
          }
        }
        frame #2 {
          n103 = invoke class="VI" method="FP.Close"() -> ()  [unwired: 3 in, 3 out]
        }
      }
      n104 = call "Update Log Path box colors.vi"("Path Ref"=w24, "Settings in"=w25) -> ()  [unwired: 8 in, 2 out]
      n105 = Unbundle By Name(w25) -> ("Log.Mode"=w21:T20, "Log.Path"=w18:path)
      n106 = To Unsigned Long Integer(number=w21) -> (unsigned 32bit integer=w20:u32)
      n107 = call "Get Timestamp Filename String.vi"() -> ("time format string"=w19:string)
      n108 = call "Add Modifier to File Name.vi"("file name modifier"=w19, "base path"=w18) -> ("appended path"=w17:path)  [unwired: 8 in, 1 out]
      n109 = Path To String(path=w18) -> (string=w27:string)
      n110 = Path To String(path=w17) -> (string=w16:string)
      n111 = local write "Log File tab control"(w20) -> ()
      n112 = property on="IO tab control" class="TabCtl (strict)"("Val(Sgnl)"=T4."Sensors" ("Value (Signaling)")) -> ()  [unwired: 2 in, 2 out]
      n113 = local write "New log file path"(w18) -> ()
      n114 = local write "Existing log file path"(w27) -> ()
      n115 = local write "Autoname new log path"(w16) -> ()
      "Host out" <- "Host"
    }
    frame Error {
    }
  }
  "error out" <- w11
  "Settings out" <- w9
  "Cancelled?" <- w8
